vi "VIH HelpGen - FILE - Symbolic Paths Collection.vi"() -> (2 "Absolute Paths":path[](array[path]), 3 "Symbolic Paths":path[](array[path]))   [LabVIEW 2014]
doc: "::: VI Helpeks :::\nCopyright (c) 2000-2026 Konstantin Shifershteyn. All rights reserved."
uses:
  <vilib>/Utility/sysdir.llb/System Directory Type.ctl
panel:
  # "VI Helpeks\nCopyright (c) 2012-2026 Konstantin Shifershteyn"
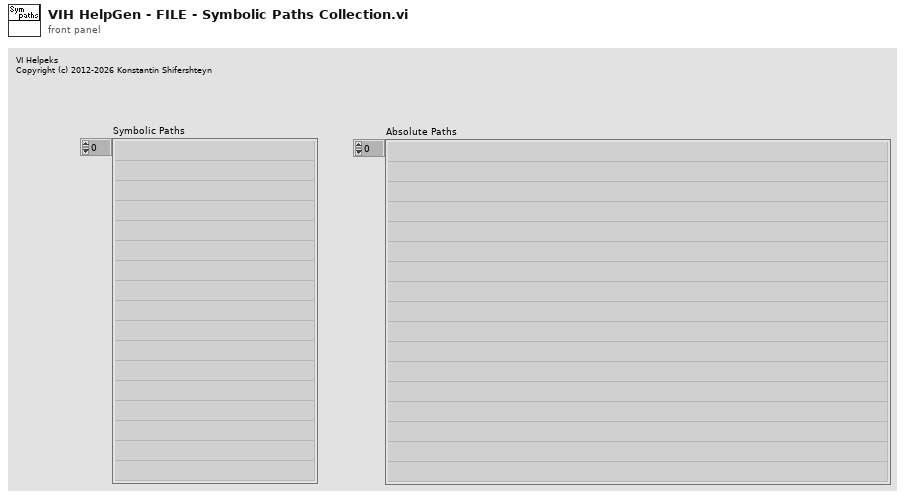
[diagram p1: front panel]
types:
  T1 = typedef "System Directory Type.ctl" = i32
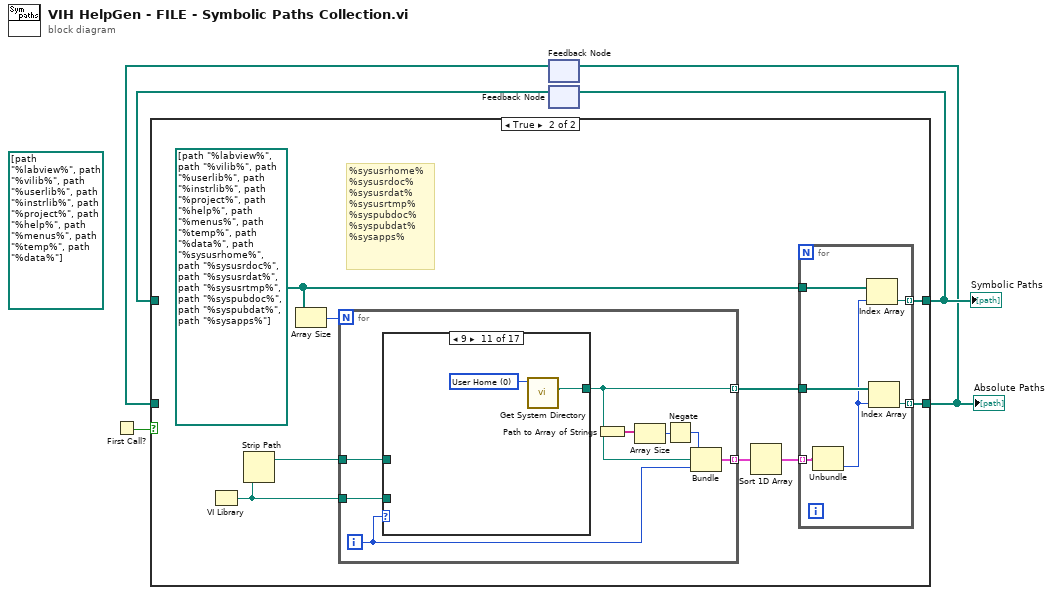
[diagram p0: block diagram]
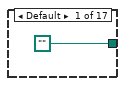
[diagram p3: hidden frame]
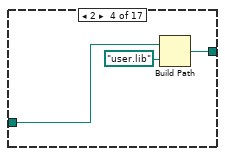
[diagram p6: hidden frame]
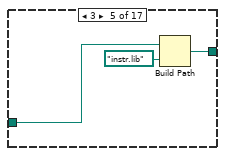
[diagram p7: hidden frame]
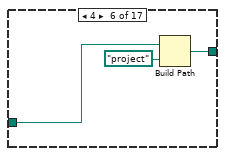
[diagram p8: hidden frame]
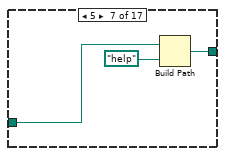
[diagram p9: hidden frame]
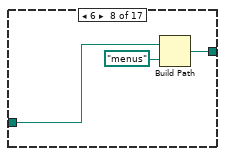
[diagram p10: hidden frame]
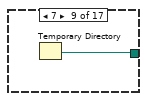
[diagram p11: hidden frame]
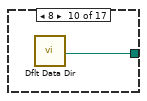
[diagram p12: hidden frame]
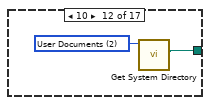
[diagram p13: hidden frame]
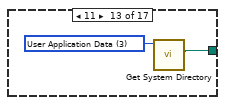
[diagram p14: hidden frame]
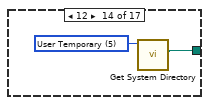
[diagram p15: hidden frame]
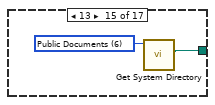
[diagram p16: hidden frame]
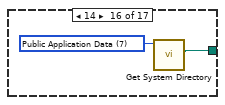
[diagram p17: hidden frame]
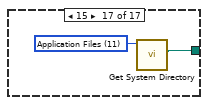
[diagram p18: hidden frame]
diagram:
  (unwired) path[] [path "%labview%", path "%vilib%", path "%userlib%", path "%instrlib%", path "%project%", path "%help%", path "%menus%", path "%temp%", path "%data%"]
  n1 = First Call?() -> (First Call?: T/F=w5:bool)
  n2 = feedback #1() -> (w1:path[])  [unwired: 1 in]
  n3 = feedback #2() -> (w3:path[])  [unwired: 1 in]
  n4 = case shown="True" w5 {
    tunnel: [w6 w14] -> w2
    tunnel: [w7 w13] -> w4
    tunnel: w3 -> [w7 _]
    tunnel: w1 -> [w6 _]
    frame False {
    }
    frame True {
      w9 = path[] [path "%labview%", path "%vilib%", path "%userlib%", path "%instrlib%", path "%project%", path "%help%", path "%menus%", path "%temp%", path "%data%", path "%sysusrhome%", path "%sysusrdoc%", path "%sysusrdat%", path "%sysusrtmp%", path "%syspubdoc%", path "%syspubdat%", path "%sysapps%"]
      # "%sysusrhome%\n%sysusrdoc%\n%sysusrdat%\n%sysusrtmp%\n%syspubdoc%\n%syspubdat%\n%sysapps%"
      n5 = VI Library() -> (path=w12:path)
      n6 = Strip Path(path=w12) -> (stripped path=w11:path)  [unwired: 1 out]
      n7 = Array Size(array=w9) -> (size(s)=w10:i32)
      n8 = for {
        N: w10 -> [_]
        tunnel: [w23] -> w15 mode=indexing
        tunnel: w12 -> [w30]
        tunnel: [w27] -> w16 mode=indexing
        tunnel: w11 -> [w26]
        i -> [w25]
        n9 = case shown="9" w25 {
          tunnel: [path "" w32 w33 w36 w39 w42 w45 w48 w49 w50 w52 w54 w56 w58 w60 w62 w64] -> w23
          tunnel: w30 -> [_ _ w33 _ _ _ _ _ _ _ _ _ _ _ _ _ _]
          tunnel: w26 -> [_ w32 _ w34 w37 w40 w43 w46 _ _ _ _ _ _ _ _ _]
          frame Default {
          }
          frame 0 {
          }
          frame 1 {
          }
          frame 2 {
            n10 = Build Path(base path=w34, name or relative path=path "user.lib") -> (appended path=w36:path)
          }
          frame 3 {
            n11 = Build Path(base path=w37, name or relative path=path "instr.lib") -> (appended path=w39:path)
          }
          frame 4 {
            n12 = Build Path(base path=w40, name or relative path=path "project") -> (appended path=w42:path)
          }
          frame 5 {
            n13 = Build Path(base path=w43, name or relative path=path "help") -> (appended path=w45:path)
          }
          frame 6 {
            n14 = Build Path(base path=w46, name or relative path=path "menus") -> (appended path=w48:path)
          }
          frame 7 {
            n15 = Temporary Directory() -> (w49:path)
          }
          frame 8 {
            n16 = call <vilib>:"Dflt Data Dir.vi"() -> ("App:Default Data Directory"=w50:path)
          }
          frame 9 {
            w51 = T1 0 items=["User Home"=0, "User Desktop"=1, "User Documents"=2, "User Application Data"=3, "User Preferences"=4, "User Temporary"=5, "Public Documents"=6, "Public Application Data"=7, "Public Preferences"=8, "Public Cache"=13, "System Core Libraries"=9, "System Installed Libraries"=10, "Application Files"=11, "Boot Volume Root"=12] ("system directory type")
            n17 = call <vilib>:"Get System Directory.vi"("system directory type"=w51) -> ("system directory"=w52:path)  [unwired: 10 in]
          }
          frame 10 {
            w53 = T1 2 items=["User Home"=0, "User Desktop"=1, "User Documents"=2, "User Application Data"=3, "User Preferences"=4, "User Temporary"=5, "Public Documents"=6, "Public Application Data"=7, "Public Preferences"=8, "Public Cache"=13, "System Core Libraries"=9, "System Installed Libraries"=10, "Application Files"=11, "Boot Volume Root"=12] ("system directory type")
            n18 = call <vilib>:"Get System Directory.vi"("system directory type"=w53) -> ("system directory"=w54:path)  [unwired: 10 in]
          }
          frame 11 {
            w55 = T1 3 items=["User Home"=0, "User Desktop"=1, "User Documents"=2, "User Application Data"=3, "User Preferences"=4, "User Temporary"=5, "Public Documents"=6, "Public Application Data"=7, "Public Preferences"=8, "Public Cache"=13, "System Core Libraries"=9, "System Installed Libraries"=10, "Application Files"=11, "Boot Volume Root"=12] ("system directory type")
            n19 = call <vilib>:"Get System Directory.vi"("system directory type"=w55) -> ("system directory"=w56:path)  [unwired: 10 in]
          }
          frame 12 {
            w57 = T1 5 items=["User Home"=0, "User Desktop"=1, "User Documents"=2, "User Application Data"=3, "User Preferences"=4, "User Temporary"=5, "Public Documents"=6, "Public Application Data"=7, "Public Preferences"=8, "Public Cache"=13, "System Core Libraries"=9, "System Installed Libraries"=10, "Application Files"=11, "Boot Volume Root"=12] ("system directory type")
            n20 = call <vilib>:"Get System Directory.vi"("system directory type"=w57) -> ("system directory"=w58:path)  [unwired: 10 in]
          }
          frame 13 {
            w59 = T1 6 items=["User Home"=0, "User Desktop"=1, "User Documents"=2, "User Application Data"=3, "User Preferences"=4, "User Temporary"=5, "Public Documents"=6, "Public Application Data"=7, "Public Preferences"=8, "Public Cache"=13, "System Core Libraries"=9, "System Installed Libraries"=10, "Application Files"=11, "Boot Volume Root"=12] ("system directory type")
            n21 = call <vilib>:"Get System Directory.vi"("system directory type"=w59) -> ("system directory"=w60:path)  [unwired: 10 in]
          }
          frame 14 {
            w61 = T1 7 items=["User Home"=0, "User Desktop"=1, "User Documents"=2, "User Application Data"=3, "User Preferences"=4, "User Temporary"=5, "Public Documents"=6, "Public Application Data"=7, "Public Preferences"=8, "Public Cache"=13, "System Core Libraries"=9, "System Installed Libraries"=10, "Application Files"=11, "Boot Volume Root"=12] ("system directory type")
            n22 = call <vilib>:"Get System Directory.vi"("system directory type"=w61) -> ("system directory"=w62:path)  [unwired: 10 in]
          }
          frame 15 {
            w63 = T1 11 items=["User Home"=0, "User Desktop"=1, "User Documents"=2, "User Application Data"=3, "User Preferences"=4, "User Temporary"=5, "Public Documents"=6, "Public Application Data"=7, "Public Preferences"=8, "Public Cache"=13, "System Core Libraries"=9, "System Installed Libraries"=10, "Application Files"=11, "Boot Volume Root"=12] ("system directory type")
            n23 = call <vilib>:"Get System Directory.vi"("system directory type"=w63) -> ("system directory"=w64:path)  [unwired: 10 in]
          }
        }
        n24 = Path to Array of Strings(0:w23) -> (2:w29:string[])  [unwired: 1 out]
        n25 = Array Size(array=w29) -> (size(s)=w28:i32)
        n26 = Negate(x=w28) -> (-x=w24:i32)
        n27 = Bundle(w24, "system directory"=w23, w25) -> (w27:cluster{i32, "system directory":path, i32})  [unwired: 1 in]
      }
      n28 = Sort 1D Array(array=w16) -> (sorted array=w8:cluster{i32, "system directory":path, i32}[])
      n29 = for {
        tunnel: w8 -> [w22] mode=indexing
        tunnel: w15 -> [w21]
        tunnel: w9 -> [w20]
        tunnel: [w19] -> w14 mode=indexing
        tunnel: [w18] -> w13 mode=indexing
        n30 = Unbundle(w22) -> (w17:i32)  [unwired: 2 out]
        n31 = Index Array(array=w20, index=w17) -> (element=w18:path)
        n32 = Index Array(array=w21, index=w17) -> (element=w19:path)
      }
    }
  }
  "Absolute Paths" <- w2
  "Symbolic Paths" <- w4
  n33 = feedback-in #1(w2) -> ()
  n34 = feedback-in #2(w4) -> ()
